vi "Latency Writer.vi"(11 "plugin gRPC address":string="localhost:51930") -> ()   [LabVIEW 2021, in "CAN_Writer_CANsub_Test_Helpers.lvlib"]
doc: "Latency test sender for the CAN writer plugin. Each frame carries its planned send time T_Out (ns, 8 bytes, big-endian) as payload. Use with Latency Reader.vi"
uses:
  CAN_Writer_CANsub_Test_Helpers.lvlib
  <vilib>/CIF Foundation/CIF XNET CAN RW/XNET CAN RW.lvclass
  <vilib>/CIF Foundation/CIF Core/CIFCore/Class/CIFCorePlugin.lvclass/CIFCorePlugin.ctl
  <vilib>/CIF Foundation/CIF Channels Core/CIFChannels/CIFChannels.lvclass
  <vilib>/CIF Foundation/CIF Core/CIFCore/Grpc/CIFCoreWrapper/CIFCoreWrapper.lvlib
  <vilib>/CIF Foundation/CIF Core/CIFCore/Class/CIFCorePlugin.lvclass
  Common/Typedef/Channels.ctl
  Common/CAN_Writer_CANsub_Common.lvlib
  Grpc/CAN_Writer_CANsub_wrapper/CAN_Writer_CANsub_Wrapper.lvlib
  <vilib>/CIF Foundation/CIF Channels Core/ChannelCommon/typedef/TimeStamps.ctl
  <vilib>/CIF Foundation/CIF Channels Core/ChannelCommon/ChannelCommon.lvlib
  <vilib>/CIF Foundation/CIF Utilities/Time/Time_CIF_U.lvlib
  <vilib>/CIF Foundation/CIF Core/CIFCore/Common/Typedef/Plugin State.ctl
  <vilib>/CIF Foundation/CIF Core/CIFCore/common/CIFCoreCommon.lvlib
  <vilib>/CIF Foundation/CIF Core/CIFCore/Common/Typedef/Timing Stats Base.ctl
  <vilib>/CIF Foundation/CIF Core/CIFCore/Common/Typedef/Timing Statistics.ctl
  <vilib>/CIF Foundation/CIF Core/CIFCore/Common/Typedef/FIFO Statistics.ctl
  <vilib>/CIF Foundation/CIF Core/CIFCore/Common/Typedef/Simple Error.ctl
  <vilib>/CIF Foundation/CIF Core/CIFCore/Common/Typedef/Monitor Doubles.ctl
  <vilib>/CIF Foundation/CIF Core/CIFCore/Common/Typedef/Monitor U64.ctl
  <vilib>/CIF Foundation/CIF Core/CIFCore/Common/Typedef/Monitor I64.ctl
  <vilib>/CIF Foundation/CIF Core/CIFCore/Common/Typedef/gRPC Reported Plugin Status.ctl
  <vilib>/xnet/xnet.llb/XNET Frame Type CAN.ctl
  <vilib>/xnet/xnet.llb/XNET Frame CAN.ctl
panel:
  out "sent":u32
  in  "period (ms)":u32=100
  in  "CAN Data":T1[](array[typedef])=[{"timestamp"=timestamp(3831573600 s since 1904-01-01), "payload"=[1, 2, 3, 4, 5, 6, 7, 8], "identifier"=512, "type"=0, "extended?"=TRUE, "echo?"=FALSE}] {"payload" format="%x"; "timestamp" format="%<%.7X\n%x>T"; "type" items=["CAN Data"=0, "CAN Remote"=1, "CAN Bus Error"=2, "CAN 2.0 Data"=8, "CAN FD Data"=16, "CAN FD+BRS Data"=24, "J1939 Data"=192, "Delay"=224, "Log Trigger"=225, "Start Trigger"=226]; "identifier" format="%x"}
  in  "Offset (ns)":i64=1000000000 format="%.0e"
  out "Node Status":T3 {"Monitor Doubles"."4" format="%#_9g"; "Monitor Doubles"."3" format="%#_9g"; "Monitor Doubles"."2" format="%#_9g"; "Monitor Doubles"."1" format="%#_9g"; "Timing Statistics (us)"."Period"."Avg" format="%_6g"}
  in  "EXIT":bool
  in  "Unload":bool
  out "error out":errorcluster
  # "Update plugin gRPC address including gRPC port and run on same target as the plugin code. \nExit will stop this VI.\nUnload will stop this VI and unload the plugin."
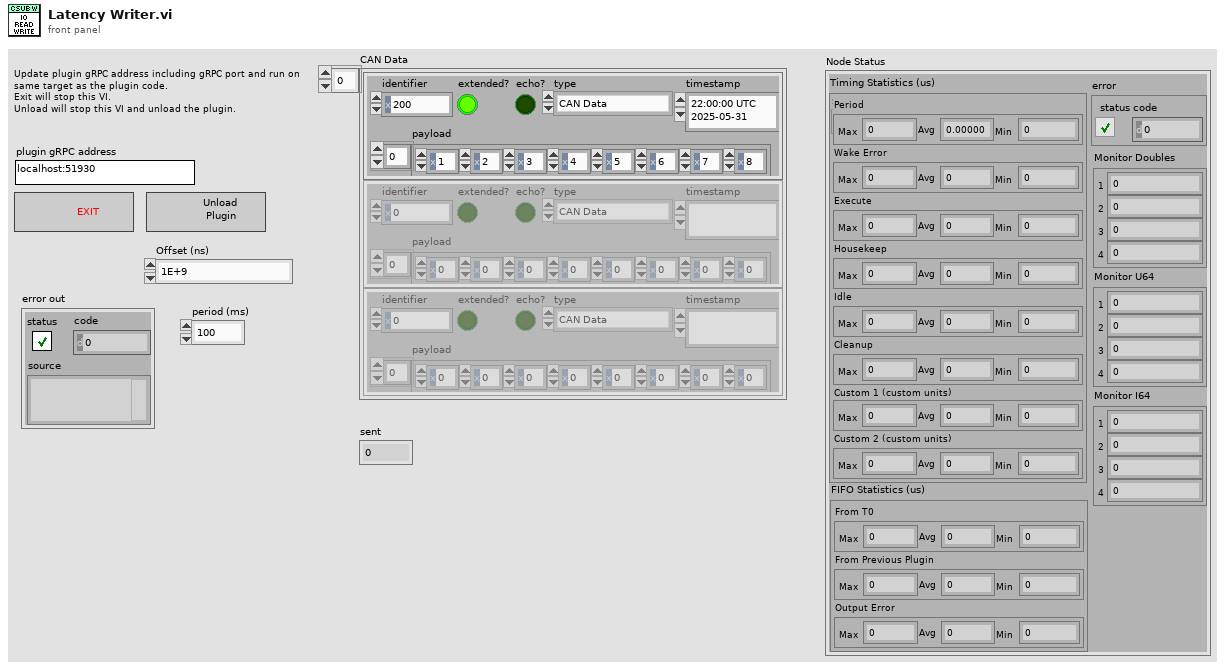
[diagram p1: front panel]
types:
  T1 = typedef "XNET Frame CAN.ctl" = cluster{"timestamp":timestamp, "payload":u8[], "identifier":u32, "type":T2, "extended?":bool, "echo?":bool}
  T2 = typedef "XNET Frame Type CAN.ctl" = u8
  T3 = typedef "CIFCoreCommon.lvlib/gRPC Reported Plugin Status.ctl" = cluster{"State":T4, "Timing Statistics (us)":T5, "FIFO Statistics (us)":T7, "error":T8, "Monitor Doubles":T9, "Monitor U64":T10, "Monitor I64":T11}
  T4 = typedef "CIFCoreCommon.lvlib/Plugin State.ctl" = enum8{"Null", "Creating", "Listening", "Running", "CleaningUp", "Destroying", "Prepared", "FTE_Run"}
  T5 = typedef "CIFCoreCommon.lvlib/Timing Statistics.ctl" = cluster{"Period":T6, "Wake Error":T6, "Execute":T6, "Housekeep":T6, "Idle":T6, "Cleanup":T6, "Custom 1 (custom units)":T6, "Custom 2 (custom units)":T6}
  T6 = typedef "CIFCoreCommon.lvlib/Timing Stats Base.ctl" = cluster{"Max":i64, "Avg":dbl, "Min":i64}
  T7 = typedef "CIFCoreCommon.lvlib/FIFO Statistics.ctl" = cluster{"From T0":T6, "From Previous Plugin":T6, "Output Error":T6}
  T8 = typedef "CIFCoreCommon.lvlib/Simple Error.ctl" = cluster{"status":bool, "code":i32}
  T9 = typedef "CIFCoreCommon.lvlib/Monitor Doubles.ctl" = cluster{"1":dbl, "2":dbl, "3":dbl, "4":dbl}
  T10 = typedef "CIFCoreCommon.lvlib/Monitor U64.ctl" = cluster{"1":u64, "2":u64, "3":u64, "4":u64}
  T11 = typedef "CIFCoreCommon.lvlib/Monitor I64.ctl" = cluster{"1":i64, "2":i64, "3":i64, "4":i64}
  T12 = typedef "grpc-lvsupport-release.lvlib/grpcId.ctl" = u64
  T13 = typedef "CIFCoreChannel_client.lvlib/cif_management_common_Channel.ctl" = cluster{"name":string, "direction":T14, "type":string, "custom_config":u8[], "connected":bool, "connected_name":string, "forced":bool, "channel_pattern":T15}
  T14 = typedef "CIFCoreChannel_client.lvlib/cif_management_common_ChannelDirection.ctl" = enum32{"CHANNELDIRECTION_UNKNOWN", "CHANNELDIRECTION_PUBLISHER", "CHANNELDIRECTION_SUBSCRIBER"}
  T15 = typedef "CIFCoreChannel_client.lvlib/cif_management_common_ChannelPattern.ctl" = enum32{"CHANNELPATTERN_UNKNOWN", "CHANNELPATTERN_TAG", "CHANNELPATTERN_FIFO", "CHANNELPATTERN_MULTIFIFO", "CHANNELPATTERN_BACKPRESSUREFIFO"}
  T16 = typedef "ChannelCommon.lvlib/TimeStamps.ctl" = cluster{"ClockID":u8, "T0":i64, "T_Out":i64}
  T17 = typedef "CAN_Writer_CANsub_Common.lvlib/Channels.ctl" = enum16{"CAN_Frames"}
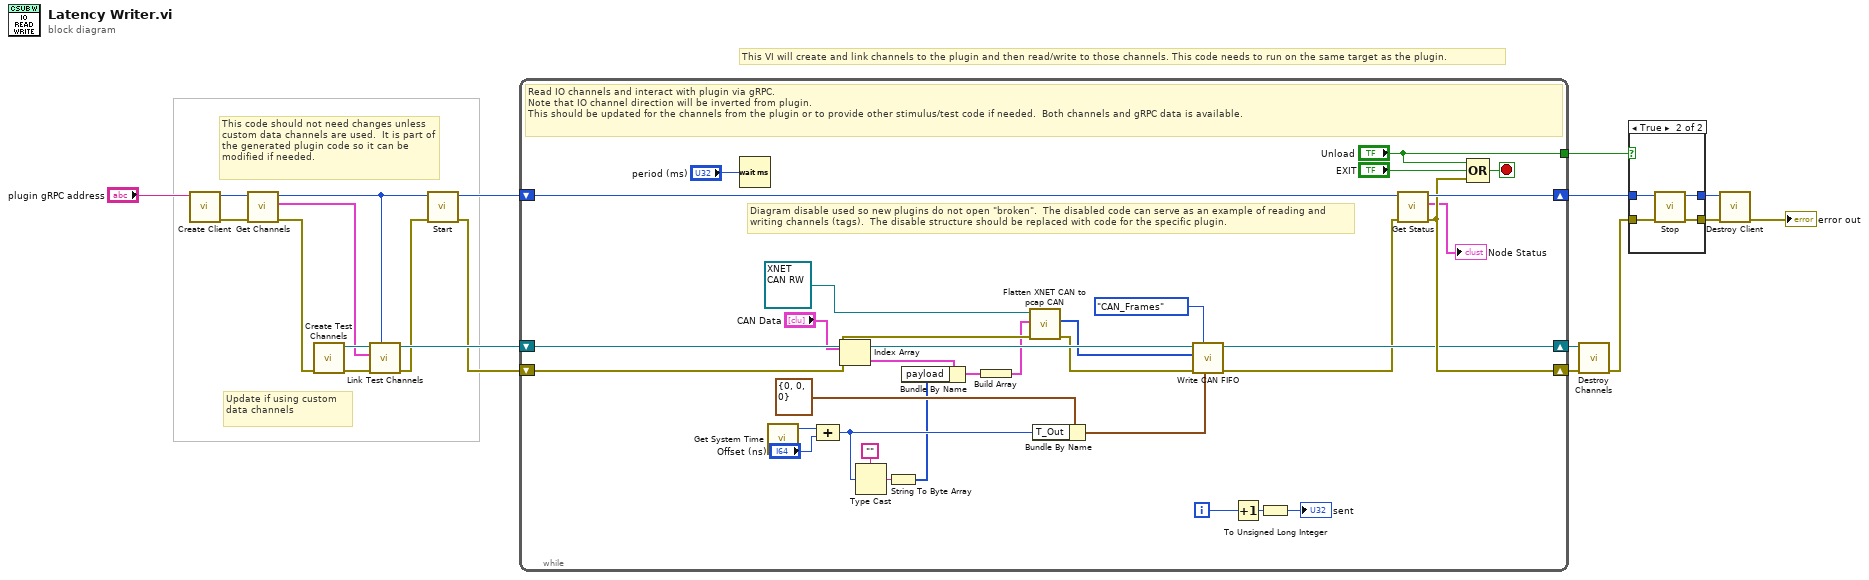
[diagram p0: block diagram]
diagram:
  # "Update if using custom data channels"
  # "This code should not need changes unless custom data channels are used.  It is part of the generated plugin code so it can be modified if needed."
  # "This VI will create and link channels to the plugin and then read/write to those channels. This code needs to run on the same target as the plugin."
  n1 = call "Create Client.vi"("address"="plugin gRPC address") -> ("error out"=w11:errorcluster, "gRPC ID Out"=w10:T12)  [unwired: 9 in]
  n2 = call <vilib>:"Get Channels.vi"("error in"=w11, "gRPC ID"=w10) -> ("error out"=w19:errorcluster, "Channels"=w15:T13[], "gRPC ID out"=w9:T12)  [unwired: 7 in]
  n3 = call "Create Test Channels.vi"("error in"=w19) -> ("error out"=w18:errorcluster, "CIFCorePlugin out"=w17:refnum<class "CIFCorePlugin.lvclass">)  [unwired: 9 in]
  n4 = call "Link Test Channels.vi"("gRPC ID in"=w9, "error in (no error)"=w18, "Channels"=w15, "CIFCorePlugin in"=w17) -> ("error out"=w7:errorcluster, "CIFCorePlugin out"=w16:refnum<class "CIFCorePlugin.lvclass">)  [unwired: 6 in]
  n5 = call <vilib>:"Start.vi"("error in"=w7, "gRPC ID"=w9) -> ("error out"=w6:errorcluster, "gRPC ID out"=w8:T12)  [unwired: 8 in]
  n6 = while {
    shift-right: [w43] -> w20
    shift-left: w16 -> [w44]
    shift-right: [w49] -> w14
    shift-left: w6 -> [w35]
    shift-right: [w50] -> w4
    shift-left: w8 -> [w51]
    tunnel: ["Unload"] -> w1
    i -> [w23]
    stop <- w48 stop-if-true
    # "Diagram disable used so new plugins do not open \"broken\".  The disabled code can serve as an example of reading and writing channels (tags).  The disable structure should be replaced with code for the specific plugin."
    # "Read IO channels and interact with plugin via gRPC.\nNote that IO channel direction will be inverted from plugin.\nThis should be updated for the channels from the plugin or to provide other stimulus/test code if needed.  Both channels and gRPC data is available."
    n7 = Wait (ms)(milliseconds to wait="period (ms)") -> ()  [unwired: 1 out]
    n8 = call <vilib>:"Get System Time.vi"() -> ("Time (ns)"=w39:i64)  [unwired: 5 in]
    n9 = Compound Arithmetic op=ADD(w39, "Offset (ns)") -> (w31:i64)
    n10 = Index Array(array="CAN Data") -> (element=w28:T1)  [unwired: 1 in]
    n11 = Type Cast(type="", x=w31) -> (*(type *) &x=w29:string)
    n12 = String To Byte Array(string=w29) -> (unsigned byte array=w24:u8[])
    n13 = Bundle By Name(cluster=w28, "payload"=w24) -> (w26:T1)
    n14 = Build Array(w26) -> (w25:T1[])
    n15 = call <vilib>:"Flatten XNET CAN to pcap CAN.vi"("error in (no error)"=w35, "XNET CAN Data"=w25, "XNET_CAN_RW in"=refnum<class "XNET CAN RW.lvclass"> refnum ("CAN_Logic in")) -> ("error out"=w34:errorcluster, "pcap CAN DATA"=w33:u8[])  [unwired: 6 in, 1 out]
    n16 = Bundle By Name(cluster=T16 {"ClockID"=0, "T0"=0, "T_Out"=0} ("FIFO Timestamps"), "T_Out"=w31) -> (w37:T16)
    n17 = call <vilib>:"Write CAN FIFO.vi"("FIFO Timestamps"=w37, "Channel Index"=Channels."CAN_Frames" ("Channels"), "error in (no error)"=w34, "Data"=w33, "CIFCorePlugin in"=w44) -> ("error out"=w42:errorcluster, "CIFCorePlugin out"=w43:refnum<class "CIFCorePlugin.lvclass">)  [unwired: 4 in, 1 out]
    n18 = Increment(x=w23) -> (x+1=w22:i32)
    n19 = To Unsigned Long Integer(number=w22) -> (unsigned 32bit integer=→"sent":u32)
    n20 = call <vilib>:"Get Status.vi"("error in"=w42, "gRPC ID"=w51) -> ("error out"=w49:errorcluster, "Node Status"=→"Node Status":T3, "gRPC ID out"=w50:T12)  [unwired: 7 in]
    n21 = Compound Arithmetic op=OR("Unload", "EXIT", w49) -> (w48:bool)
  }
  n22 = call <vilib>:"Destroy Channels.vi"("error in (no error)"=w14, "CIFCorePlugin in"=w20) -> ("error out"=w5:errorcluster)  [unwired: 7 in, 2 out]
  n23 = case shown="True" w1 {
    tunnel: w5 -> [w52 w57]
    tunnel: w4 -> [w53 w56]
    tunnel: [w53 w55] -> w3
    tunnel: [w52 w54] -> w2
    frame False {
    }
    frame True {
      n24 = call <vilib>:"Stop.vi"("error in"=w57, "gRPC ID"=w56) -> ("error out"=w54:errorcluster, "gRPC ID out"=w55:T12)  [unwired: 8 in]
    }
  }
  n25 = call "Destroy Client.vi"("error in"=w2, "gRPC ID"=w3) -> ("error out"=→"error out":errorcluster)  [unwired: 9 in]
